vi "UI - Initiate Connection.vi"(8 "error in (no error)":errorcluster, 9 "Controller Address 2":string, 10 "Controller Address":string, 11 "Message Queue":refnum<queue>) -> (0 "error out":errorcluster, 1 "Connected?":bool)   [LabVIEW 2025]
uses:
  Globals/Global - Configuration Options.vi
  Message Queue/Message Queue.lvlib
  controls/Control State.ctl
  controls/Variable References.ctl
  Globals/Global - UI Stream and Variable Connections.vi
  Message Queue/Message Cluster.ctl
  controls/IO References.ctl
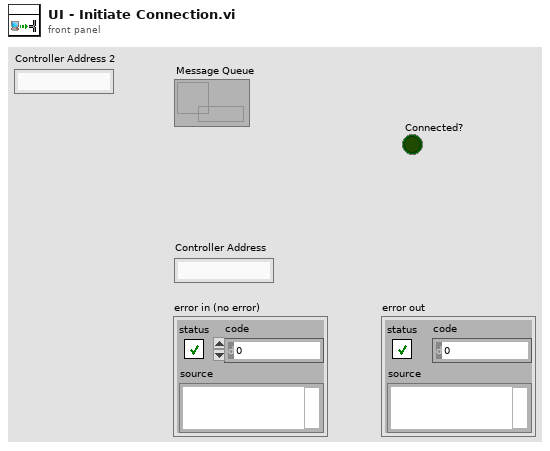
[diagram p1: front panel]
types:
  T1 = typedef "Control State.ctl" = enum16{"Safe State", "Control (PID)"}
  T2 = typedef "Message Queue.lvlib/Message Cluster.ctl" = cluster{"Message":string, "Message Data":variant}
  T3 = typedef "IO References.ctl" = cluster{"Control Input Values":refnum<k21>[], "Control Output Values":refnum<k21>[], "Temperature Values":refnum<k21>[], "Threshold Exceeded":refnum<k21>, "Control Input Values 2":refnum<k21>[], "Control Output Values 2":refnum<k21>[], "Control Digital Values":refnum<k21>[], "Control Digital Values 2":refnum<k21>[]}
  T4 = typedef "Variable References.ctl" = cluster{"CPU Usage":refnum<k21>, "Contiguous Memory":refnum<k21>, "Control Mode":refnum<k21>, "Control Loop Period":refnum<k21>, "Low Speed Loop Period":refnum<k21>, "CPU Usage crio 2":refnum<k21>}
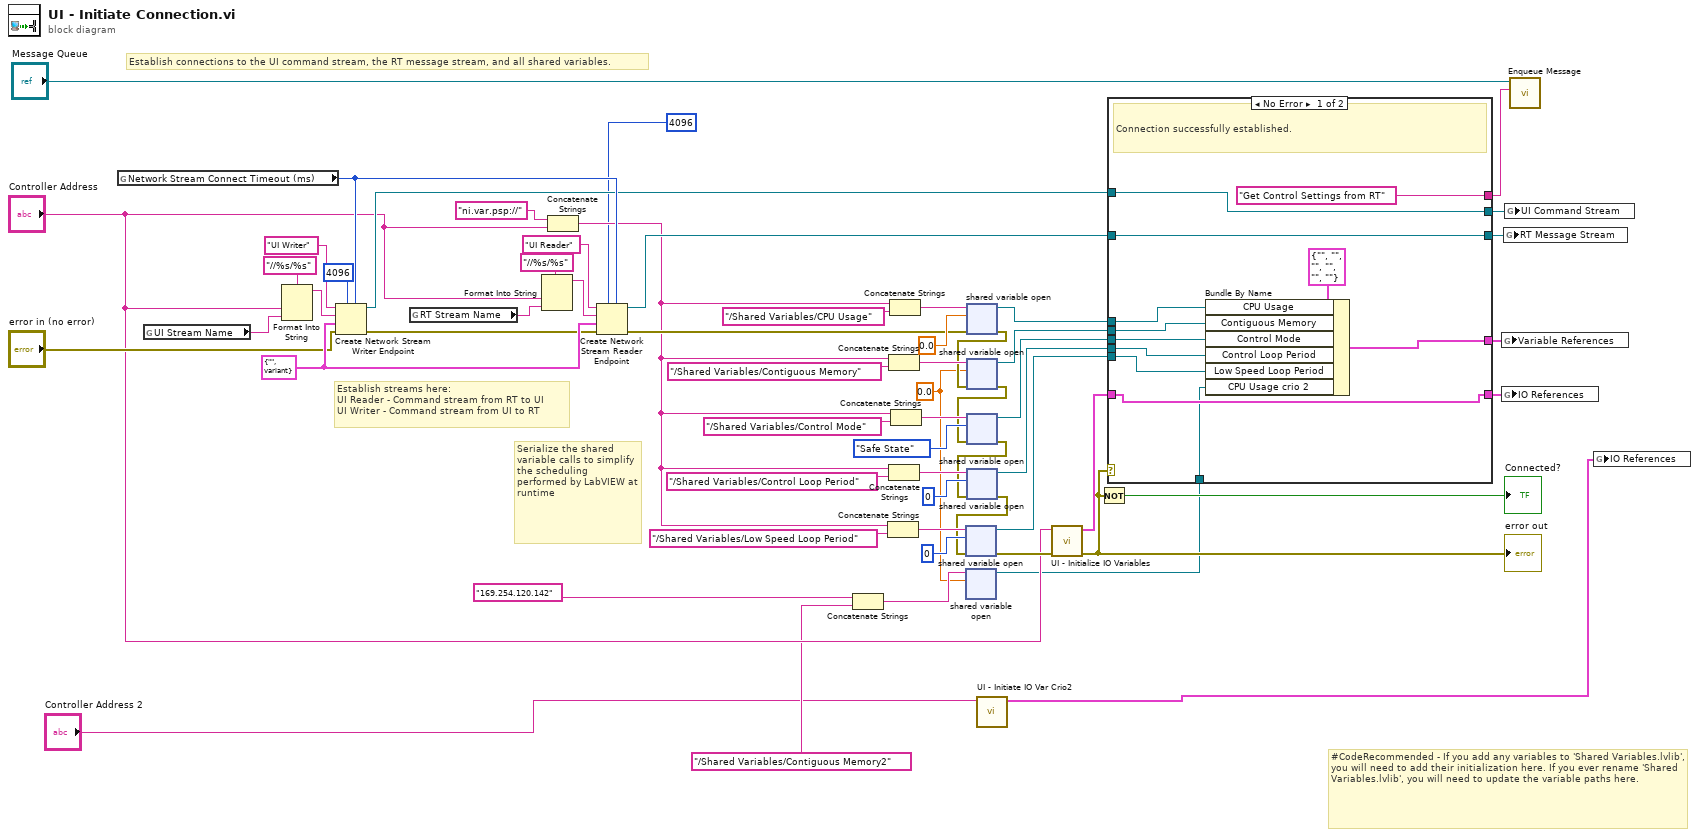
[diagram p0: block diagram]
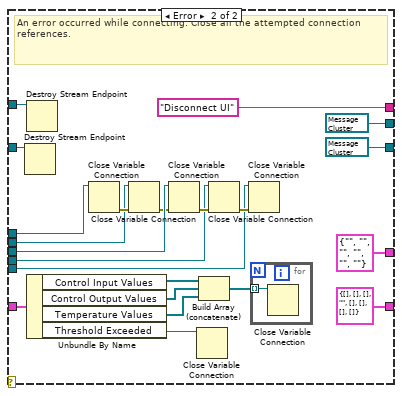
[diagram p2: hidden frame]
diagram:
  w5 = 0.0
  w51 = T2 {"Message"="", "Message Data"=variant} ("Message Cluster")
  # "Establish connections to the UI command stream, the RT message stream, and all shared variables."
  # "#CodeRecommended - If you add any variables to 'Shared Variables.lvlib', you will need to add their initialization here. If you ever rename 'Shared Variables.lvlib', you will need to update the variable paths here."
  # "Establish streams here:\nUI Reader - Command stream from RT to UI\nUI Writer - Command stream from UI to RT"
  # "Serialize the shared variable calls to simplify the scheduling performed by LabVIEW at runtime"
  n1 = global read "Global - Configuration Options.vi" "Network Stream Connect Timeout (ms)"() -> (w50:i32)
  n2 = global read "Global - Configuration Options.vi" "UI Stream Name"() -> (w58:string)
  n3 = Format Into String(format string="//%s/%s", "Controller Address", w58) -> (resulting string=w57:string)  [unwired: 2 in, 1 out]
  n4 = Create Network Stream Writer Endpoint(5:w50, 7:4096 ("writer buffer size"), 8:"error in (no error)", 9:w51, 10:w57, 11:"UI Writer" ("writer name")) -> (0:w23:errorcluster, 3:w31:refnum<k21>)  [unwired: 1 in]
  n5 = global read "Global - Configuration Options.vi" "RT Stream Name"() -> (w55:string)
  n6 = Format Into String(format string="//%s/%s", "Controller Address", w55) -> (resulting string=w54:string)  [unwired: 2 in, 1 out]
  n7 = Concatenate Strings("ni.var.psp://", "Controller Address") -> (w16:string)
  n8 = Create Network Stream Reader Endpoint(5:w50, 7:4096 ("reader buffer size"), 8:w23, 9:w51, 10:w54, 11:"UI Reader" ("reader name")) -> (0:w22:errorcluster, 3:w30:refnum<k21>)  [unwired: 1 in]
  n9 = Concatenate Strings("169.254.120.142" ("Controller Address 2"), "/Shared Variables/Contiguous Memory2") -> (w6:string)
  n10 = Concatenate Strings(w16, "/Shared Variables/Low Speed Loop Period") -> (w20:string)
  n11 = Concatenate Strings(w16, "/Shared Variables/Contiguous Memory") -> (w44:string)
  n12 = Concatenate Strings(w16, "/Shared Variables/Control Loop Period") -> (w40:string)
  n13 = Concatenate Strings(w16, "/Shared Variables/CPU Usage") -> (w47:string)
  n14 = Concatenate Strings(w16, "/Shared Variables/Control Mode") -> (w43:string)
  n15 = shared-variable-open(w6, w5) -> (w4:refnum<k21>)  [unwired: 2 in, 1 out]
  n16 = shared-variable-open(w47, w22, 0.0) -> (w35:refnum<k21>, w37:errorcluster)  [unwired: 1 in]
  n17 = shared-variable-open(w44, w37, w5) -> (w34:refnum<k21>, w15:errorcluster)  [unwired: 1 in]
  n18 = shared-variable-open(w43, w15, Control_State."Safe State" ("FPGA State")) -> (w33:refnum<k21>, w36:errorcluster)  [unwired: 1 in]
  n19 = shared-variable-open(w40, w36, u32 0) -> (w32:refnum<k21>, w19:errorcluster)  [unwired: 1 in]
  n20 = shared-variable-open(w20, w19, u32 0) -> (w18:refnum<k21>, w13:errorcluster)  [unwired: 1 in]
  n21 = call "UI - Initiate IO Var Crio2.vi"("Controller Address"="Controller Address 2") -> ("IO References"=w1:T3)  [unwired: 10 in]
  n22 = call "UI - Initialize IO Variables.vi"("error in (no error)"=w13, "Controller Address"="Controller Address") -> ("error out"=w12:errorcluster, "IO References"=w2:T3)  [unwired: 8 in]
  "error out" <- w12
  n23 = Not(x=w12) -> (.not. x?=→"Connected?":bool)
  n24 = case shown="No Error" w12 {
    tunnel: w35 -> [w71 w90]
    tunnel: w34 -> [w70 w87]
    tunnel: w33 -> [w69 w88]
    tunnel: w32 -> [w68 w89]
    tunnel: w31 -> [w64 w93]
    tunnel: w30 -> [w66 w94]
    tunnel: [w67 T4 {"CPU Usage"="", "Contiguous Memory"="", "Control Mode"="", "Control Loop Period"="", "Low Speed Loop Period"="", "CPU Usage crio 2"=""} ("Variable References")] -> w29
    tunnel: [w66 refnum<k21> refnum] -> w28
    tunnel: [w64 refnum<k21> refnum] -> w27
    tunnel: ["Get Control Settings from RT" "Disconnect UI"] -> w25
    tunnel: w18 -> [w63 w81]
    tunnel: [w62 T3 {"Control Input Values"=[], "Control Output Values"=[], "Temperature Values"=[], "Threshold Exceeded"="", "Control Input Values 2"=[], "Control Output Values 2"=[], "Control Digital Values"=[], "Control Digital Values 2"=[]} ("IO References")] -> w14
    tunnel: w2 -> [w62 w78]
    tunnel: w4 -> [w61 _]
    frame No Error {
      # "Connection successfully established."
      n25 = Bundle By Name(cluster=T4 {"CPU Usage"="", "Contiguous Memory"="", "Control Mode"="", "Control Loop Period"="", "Low Speed Loop Period"="", "CPU Usage crio 2"=""} ("Variable References"), "CPU Usage"=w71, "Contiguous Memory"=w70, "Control Mode"=w69, "Control Loop Period"=w68, "Low Speed Loop Period"=w63, "CPU Usage crio 2"=w61) -> (w67:T4)
    }
    frame Error {
      # "An error occurred while connecting. Close all the attempted connection references."
      n26 = Destroy Stream Endpoint(11:w94) -> ()  [unwired: 1 in, 1 out]
      n27 = Destroy Stream Endpoint(11:w93) -> ()  [unwired: 1 in, 1 out]
      n28 = Unbundle By Name(w78) -> ("Control Input Values"=w77:refnum<k21>[], "Control Output Values"=w76:refnum<k21>[], "Temperature Values"=w75:refnum<k21>[], "Threshold Exceeded"=w73:refnum<k21>)
      n29 = Close Variable Connection(11:w90) -> (0:w91:errorcluster)  [unwired: 1 in]
      n30 = Close Variable Connection(8:w91, 11:w87) -> (0:w80:errorcluster)
      n31 = Close Variable Connection(8:w80, 11:w88) -> (0:w92:errorcluster)
      n32 = Close Variable Connection(11:w73) -> ()  [unwired: 1 in, 1 out]
      n33 = Build Array (concatenate)(w77, w76, w75) -> (w74:refnum<k21>[])
      n34 = Close Variable Connection(8:w92, 11:w89) -> (0:w82:errorcluster)
      n35 = Close Variable Connection(8:w82, 11:w81) -> ()  [unwired: 1 out]
      n36 = for {
        tunnel: w74 -> [w95] mode=indexing
        n37 = Close Variable Connection(11:w95) -> ()  [unwired: 1 in, 1 out]
      }
    }
  }
  n38 = global write "Global - UI Stream and Variable Connections.vi" "Variable References"(w29) -> ()
  n39 = global write "Global - UI Stream and Variable Connections.vi" "IO References"(w14) -> ()
  n40 = global write "Global - UI Stream and Variable Connections.vi" "RT Message Stream"(w28) -> ()
  n41 = global write "Global - UI Stream and Variable Connections.vi" "UI Command Stream"(w27) -> ()
  n42 = call "Enqueue Message.vi"("Message"=w25, "Message Queue"="Message Queue") -> ()  [unwired: 8 in, 2 out]
  n43 = global write "Global - UI Stream and Variable Connections.vi" "IO References"(w1) -> ()
